vi "getMasksIntB.vi"(0 "dl in":refnum<class "dl.lvclass">, 1 "maskCounts":i32[](array[numeric]), 5 "error in (no error)":errorcluster) -> (14 "dl out":refnum<class "dl.lvclass">, 15 "Vertices":T3[](array[typedef]), 16 "total vertices":i32, 17 "verticesPerPolygons":i32[](array[numeric]), 18 "BatchMasks":T1[](array[typedef]), 19 "error out":errorcluster)   [LabVIEW 2025, in "dl.lvlib" / "dl.lvclass"]
doc: "Parse Segmentation Results (Masks)\n\nInput:\n- `maskCounts`: Number of detected segmentation masks per image, returned by `runDetectionB`.\n\nOutputs:\n- `Vertices`: Flattened 1D array containing the vertices of all detected masks across the batch.\n- `totalVertices`: Total number of vertices across all detected masks in the batch.\n- `verticesPerPolygons`: Number of vertices in each polygon.\n- `BatchMasks`: Segmentation results organized by image, with each image containing its own array of polygons."
uses:
  dl.lvclass
  LVPointInt.ctl
  def/ImageMasks.ctl
  def/Polygon.ctl
  dl.lvclass/dl.ctl
  def/Mask.ctl
  cc241279-2497-45f2-9759-cbad2faff15f.vi
  253f3596-1e81-40e0-a631-691f5b1a1e14.vi
  tcv/tcv.lvclass
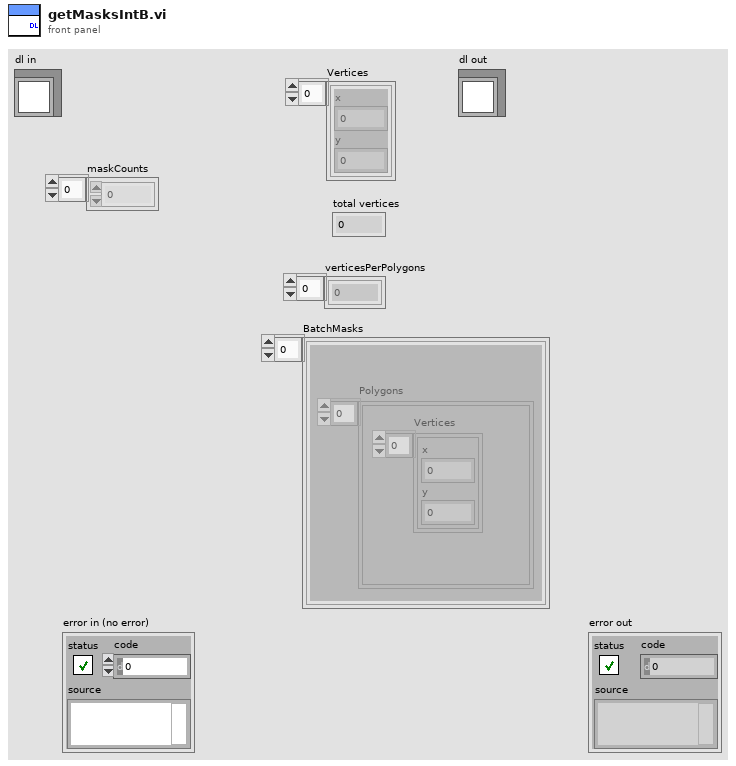
[diagram p1: front panel]
types:
  T1 = typedef "dl.lvlib/dl.lvclass/ImageMasks.ctl" = cluster{"Polygons ":T2[]}
  T2 = typedef "dl.lvlib/dl.lvclass/Polygon.ctl" = cluster{"Vertices":T3[]}
  T3 = typedef "dl.lvlib/dl.lvclass/LVPointInt.ctl" = cluster{"x":i32, "y":i32}
  T4 = typedef "dl.lvlib/dl.lvclass/Mask.ctl" = cluster{"Polygons":T2[]}
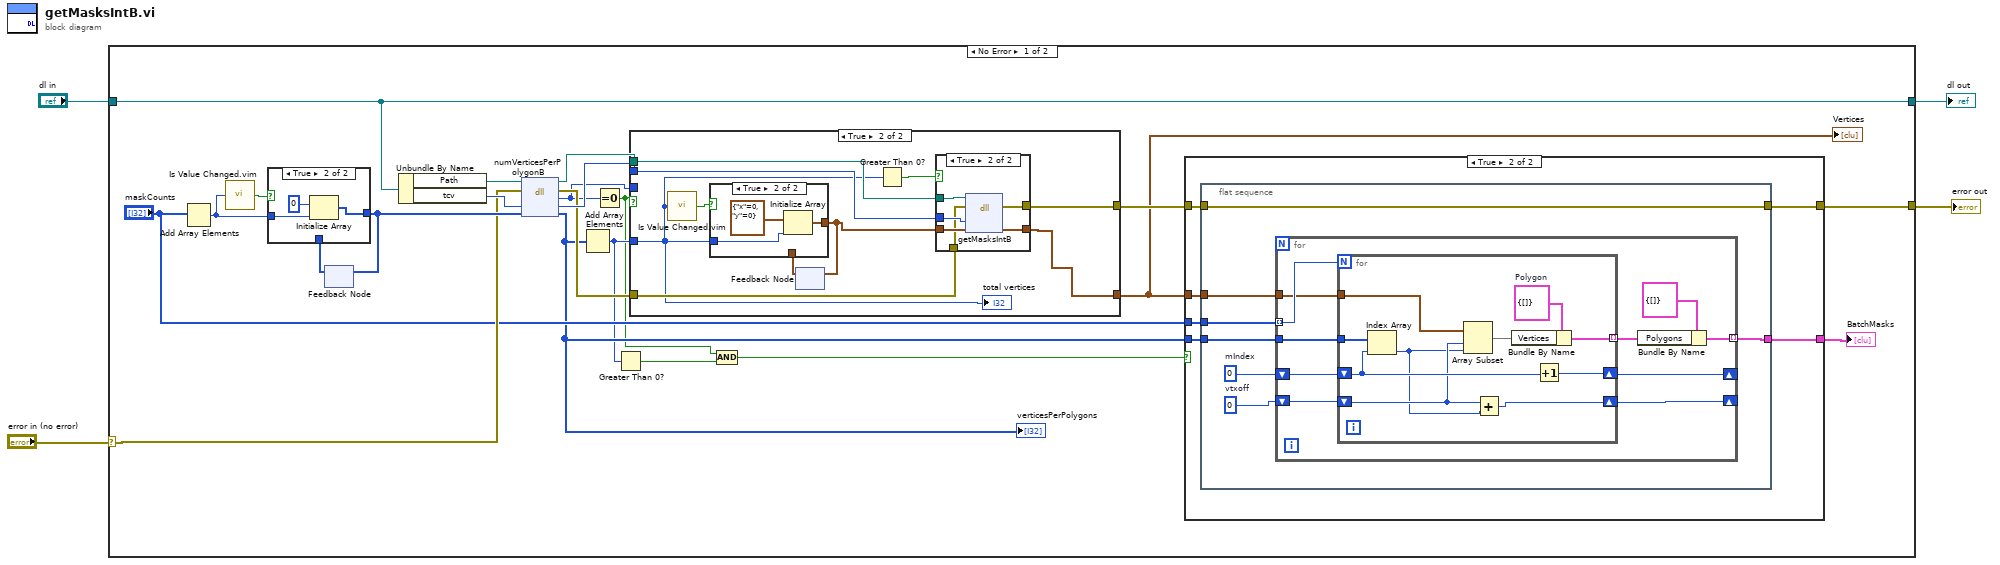
[diagram p0: block diagram]
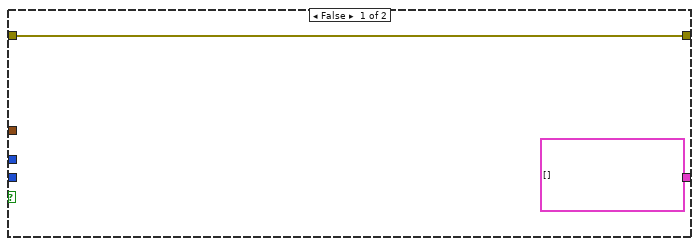
[diagram p2: hidden frame]
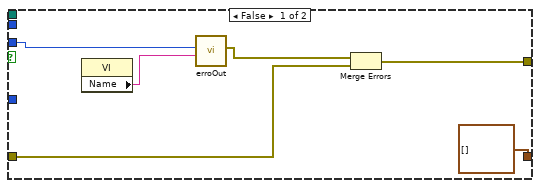
[diagram p3: hidden frame]
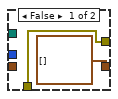
[diagram p4: hidden frame]
diagram:
  n1 = case shown="No Error" "error in (no error)" {
    selector: "error in (no error)" -> [w17 w95]
    tunnel: [w13 w95] -> w3
    tunnel: [w23 w94] -> w1
    tunnel: "dl in" -> [w23 w94]
    frame No Error {
      n2 = Add Array Elements(numeric array="maskCounts") -> (sum=w26:i32)
      n3 = call "Is Value Changed.vim"("value"=w26) -> ("changed or first call?"=w25:bool)
      n4 = feedback #1() -> (w24:i32[])  [unwired: 1 in]
      n5 = case shown="True" w25 {
        tunnel: w26 -> [_ w92]
        tunnel: [w90 w91] -> w20
        tunnel: w24 -> [w90 _]
        frame False {
        }
        frame True {
          n6 = Initialize Array(0, w92) -> (w91:i32[])
        }
      }
      n7 = feedback-in #1(w20) -> ()
      n8 = Unbundle By Name(w23) -> ("Path"=w22:path, "tcv"=w21:u64)
      n9 = dll-call lib="D:/Test/adslvPackageDev/Resources/TCV_Lib.dll" fn="numVerticesPerPolygonB"(path in=w22, error in=w17, "tcv"=w21, "verticesPerPolygons"=w20) -> (path out=w19:path, error out=w16:errorcluster, "succNVPP"=w15:i32, "tcv"=w18:u64, "verticesPerPolygons"=w11:i32[])  [unwired: 1 in]
      "verticesPerPolygons" <- w11
      n10 = Add Array Elements(numeric array=w11) -> (sum=w10:i32)
      n11 = Equal To 0?(x=w15) -> (x = 0?=w8:bool)
      n12 = Greater Than 0?(x=w10) -> (x > 0?=w9:bool)
      n13 = case shown="True" w8 {
        tunnel: w10 -> [_ w69]
        tunnel: w19 -> [_ w74]
        tunnel: w18 -> [_ w73]
        tunnel: w16 -> [w64 w71]
        tunnel: [w63 w70] -> w14
        tunnel: w15 -> [w67 _]
        tunnel: [T3[] [] ("VerticesBufferI") w68] -> w6
        frame False {
          n14 = property class="VI"() -> ("Name"=w66:string)  [unwired: 2 in, 2 out]
          n15 = call "erroOut.vi"("source"=w66, "code"=w67) -> ("output cluster"=w65:errorcluster)  [unwired: 9 in]
          n16 = Merge Errors(w65, w64) -> (w63:errorcluster)
        }
        frame True {
          n17 = call "Is Value Changed.vim"("value"=w69) -> ("changed or first call?"=w77:bool)
          n18 = feedback #2() -> (w76:T3[])  [unwired: 1 in]
          n19 = case shown="True" w77 {
            tunnel: w69 -> [_ w88]
            tunnel: [w86 w87] -> w72
            tunnel: w76 -> [w86 _]
            frame False {
            }
            frame True {
              n20 = Initialize Array(T3 {"x"=0, "y"=0} ("LVPointInt"), w88) -> (w87:T3[])
            }
          }
          n21 = feedback-in #2(w72) -> ()
          n22 = Greater Than 0?(x=w69) -> (x > 0?=w75:bool)
          n23 = case shown="True" w75 {
            tunnel: w74 -> [_ w85]
            tunnel: w73 -> [_ w84]
            tunnel: w72 -> [_ w83]
            tunnel: [T3[] [] ("VerticesBufferI") w82] -> w68
            tunnel: w71 -> [w78 w81]
            tunnel: [w78 w80] -> w70
            frame False {
            }
            frame True {
              n24 = dll-call lib="D:/Test/adslvPackageDev/Resources/TCV_Lib.dll" fn="getMasksIntB"(path in=w85, error in=w81, "tcv"=w84, "VerticesBufferI"=w83) -> (error out=w80:errorcluster, "VerticesBufferI"=w82:T3[])  [unwired: 3 in, 1 out]
            }
          }
          "total vertices" <- w69
        }
      }
      "Vertices" <- w6
      n25 = And(x=w8, y=w9) -> (x .and. y?=w7:bool)
      n26 = case shown="True" w7 {
        tunnel: w14 -> [w27 w34]
        tunnel: [w27 w33] -> w13
        tunnel: "maskCounts" -> [_ w32]
        tunnel: w11 -> [_ w31]
        tunnel: w6 -> [_ w30]
        tunnel: [T4[] [] w29] -> w5
        frame False {
        }
        frame True {
          n27 = flat-sequence {
            tunnel: w34 -> [w41]
            tunnel: [w41] -> w33
            tunnel: w32 -> [w40]
            tunnel: w31 -> [w37]
            tunnel: w30 -> [w36]
            tunnel: [w35] -> w29
            frame #0 {
              w38 = 0  # vtxoff
              w39 = 0  # mIndex
              n28 = for {
                tunnel: w40 -> [w51] mode=indexing
                shift-right: [w46] -> _
                shift-left: w39 -> [w49]
                shift-right: [w45] -> _
                shift-left: w38 -> [w47]
                tunnel: w37 -> [w50]
                tunnel: w36 -> [w48]
                tunnel: [w43] -> w35 mode=indexing
                n29 = for {
                  N: w51 -> [_]
                  tunnel: w50 -> [w61]
                  shift-right: [w59] -> w46
                  shift-left: w49 -> [w60]
                  shift-right: [w54] -> w45
                  shift-left: w47 -> [w56]
                  tunnel: w48 -> [w57]
                  tunnel: [w52] -> w44 mode=indexing
                  w58 = T2 {"Vertices"=[]}  # Polygon
                  n30 = Index Array(array=w61, index=w60) -> (element=w55:i32)
                  n31 = Array Subset(array=w57, index=w56, length=w55) -> (w53:T3[])
                  n32 = Add(x=w56, y=w55) -> (x+y=w54:i32)
                  n33 = Bundle By Name(cluster=w58, "Vertices"=w53) -> (w52:T2)
                  n34 = Increment(x=w60) -> (x+1=w59:i32)
                }
                n35 = Bundle By Name(cluster=T1 {"Polygons "=[]} ("ImageMasks"), "Polygons"=w44) -> (w43:T1)
              }
            }
          }
        }
      }
      "BatchMasks" <- w5
    }
    frame Error {
    }
  }
  "error out" <- w3
  "dl out" <- w1
